vi "Unregister.vi"(8 "error in (no error)":errorcluster, 11 "handler name":string) -> (0 "error out":errorcluster)   [LabVIEW 2018, in "GLog.lvlib" / "UI Updater.lvlib"]
uses:
  UI Updater.lvlib
  Events/Unregister.ctl
  Unregister Response Data.ctl
  UI Updater Global.vi
panel:
  # "Connector Pane"
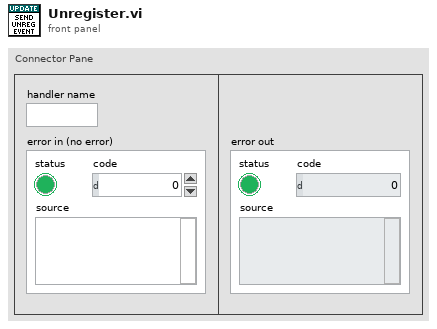
[diagram p1: front panel]
types:
  T1 = typedef "GLog.lvlib/UI Updater.lvlib/Unregister Response Data.ctl" = cluster{"last call?":bool}
  T2 = typedef "GLog.lvlib/UI Updater.lvlib/Unregister.ctl" = cluster{"handler name":string, "response notifier":refnum<notifier>}
  T3 = typedef "GLog.lvlib/UI Updater.lvlib/Events.ctl" = cluster{"Write Log":refnum<user-event>, "Register":refnum<user-event>, "Unregister":refnum<user-event>}
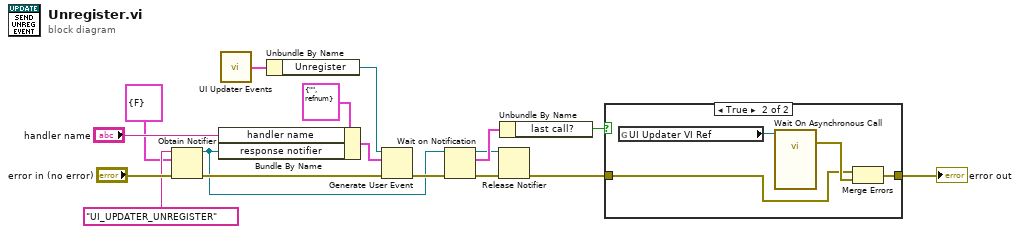
[diagram p0: block diagram]
diagram:
  n1 = Obtain Notifier(name (unnamed)="UI_UPDATER_UNREGISTER", notification data type=T1 {"last call?"=FALSE} ("unregister response data"), error in (no error)="error in (no error)") -> (notifier out=w8:refnum<notifier>, error out=w11:errorcluster)  [unwired: 1 in, 1 out]
  n2 = Bundle By Name(cluster=T2 {"handler name"="", "response notifier"=refnum} ("event data"), "handler name"="handler name", "response notifier"=w8) -> (w13:T2)
  n3 = call "UI Updater Events.vi"() -> ("UI Updater"=w14:T3)  [unwired: 1 in]
  n4 = Unbundle By Name(w14) -> ("Unregister"=w15:refnum<user-event>)
  n5 = Generate User Event(user event=w15, event data cluster=w13, error in=w11) -> (error out=w9:errorcluster)  [unwired: 1 in, 1 out]
  n6 = Wait on Notification(notifier=w8, error in (no error)=w9) -> (notifier out=w4:refnum<notifier>, notification=w6:T1, error out=w3:errorcluster)  [unwired: 2 in, 1 out]
  n7 = Release Notifier(notifier=w4, error in (no error)=w3) -> (error out=w1:errorcluster)  [unwired: 1 in, 2 out]
  n8 = Unbundle By Name(w6) -> ("last call?"=w5:bool)
  n9 = case shown="True" w5 {
    tunnel: [w18 w20] -> w2
    tunnel: w1 -> [w18 w19]
    frame False {
    }
    frame True {
      n10 = global read "UI Updater Global.vi" "UI Updater VI Ref"() -> (w22:refnum<vi>)
      n11 = call-by-ref "Wait On Asynchronous Call"(reference=w22) -> (error out=w21:errorcluster)  [unwired: 13 in, 1 out]
      n12 = Merge Errors(w19, w21) -> (w20:errorcluster)
    }
  }
  "error out" <- w2
